vi "Create UNSUBSCRIBE Packet.vi"(5 "UNSUBSCRIBE in":refnum<class "UNSUBSCRIBE.lvclass">, 8 "error in (no error)":errorcluster, 9 "Packet ID (0: generate new)":u16 format="%04x", 11 "Topic Subscriptions":string[](array[string])) -> (0 "error out":errorcluster, 2 "Bytes Stream":u8[](array[numeric]) format="%08b", 3 "UNSUBSCRIBE out":refnum<class "UNSUBSCRIBE.lvclass">)   [LabVIEW 2013, in "MQTT_Control_Packets.lvlib" / "UNSUBSCRIBE.lvclass"]
uses:
  UNSUBSCRIBE.lvclass
  ControlPacket/ControlPacket.lvclass/ControlPacket.ctl
  ControlPacket/ControlPacket.lvclass
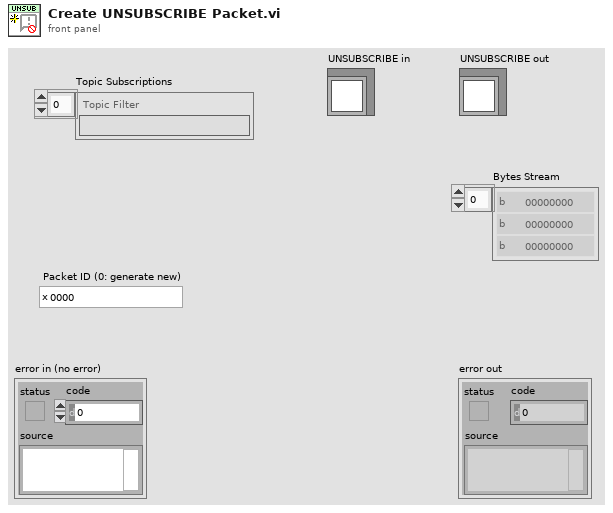
[diagram p1: front panel]
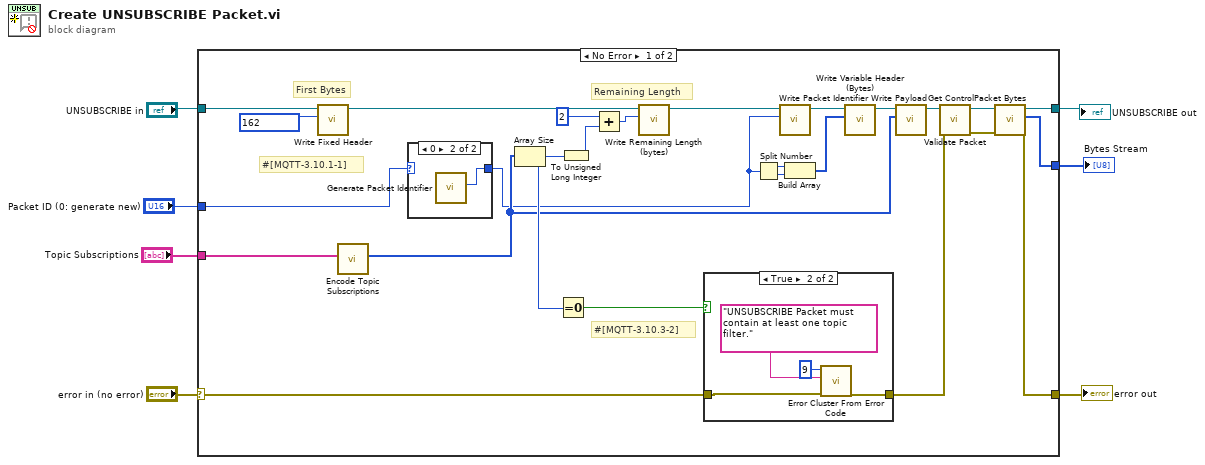
[diagram p0: block diagram]
diagram:
  n1 = case shown="No Error" "error in (no error)" {
    selector: "error in (no error)" -> [w20 w42]
    tunnel: [w9 w42] -> w3
    tunnel: [w11 w41] -> w2
    tunnel: "UNSUBSCRIBE in" -> [w33 w41]
    tunnel: "Packet ID (0: generate new)" -> [w14 _]
    tunnel: "Topic Subscriptions" -> [w16 _]
    tunnel: [w8 _] -> w1
    frame No Error {
      # "#[MQTT-3.10.3-2]"
      # "#[MQTT-3.10.1-1]"
      # "Remaining Length"
      # "First Bytes"
      n2 = call "Write Fixed Header.vi"("Fixed Header"=u8 162, "ControlPacket in"=w33) -> ("ControlPacket out"=w32:refnum<class "UNSUBSCRIBE.lvclass">)  [unwired: 9 in]
      n3 = call "Encode Topic Subscriptions.vi"("Topic Subscriptions"=w16) -> ("Length-Prefixed Field"=w15:u8[])  [unwired: 10 in]
      n4 = case shown="0" w14 {
        selector: w14 -> [w34 _]
        tunnel: [w34 w35] -> w13
        frame Default {
        }
        frame 0 {
          n5 = call "Generate Packet Identifier.vi"() -> ("Packet Identifier"=w35:u16)  [unwired: 11 in]
        }
      }
      n6 = Array Size(array=w15) -> (size(s)=w21:i32)
      n7 = Equal To 0?(x=w21) -> (x = 0?=w19:bool)
      n8 = To Unsigned Long Integer(number=w21) -> (unsigned 32bit integer=w22:u32)
      n9 = Add(x=u32 2 ("Remaining Length (bytes)"), y=w22) -> (x+y=w24:u32)
      n10 = call "Write Remaining Length (bytes).vi"("Remaining Length (bytes)"=w24, "ControlPacket in"=w32) -> ("ControlPacket out"=w28:refnum<class "UNSUBSCRIBE.lvclass">)  [unwired: 9 in]
      n11 = case shown="True" w19 {
        tunnel: w20 -> [w36 w39]
        tunnel: [w36 w40] -> w17
        frame False {
        }
        frame True {
          n12 = call <vilib>:"Error Cluster From Error Code.vi"("error in (no error)"=w39, "error message (\"\")"="UNSUBSCRIBE Packet must contain at least one topic filter.", "error code (0)"=9) -> ("error out"=w40:errorcluster)  [unwired: 6 in]
        }
      }
      n13 = Split Number(x=w13) -> (hi(x)=w31:u8, lo(x)=w30:u8)
      n14 = call "Write Packet Identifier.vi"("Packet Identifier"=w13, "ControlPacket in"=w28) -> ("ControlPacket out"=w27:refnum<class "UNSUBSCRIBE.lvclass">)  [unwired: 9 in]
      n15 = Build Array(w31, w30) -> (w29:u8[])
      n16 = call "Write Variable Header (Bytes).vi"("Variable Header (Bytes)"=w29, "ControlPacket in"=w27) -> ("ControlPacket out"=w23:refnum<class "UNSUBSCRIBE.lvclass">)  [unwired: 9 in]
      n17 = call "Write Payload.vi"("Payload"=w15, "ControlPacket in"=w23) -> ("ControlPacket out"=w18:refnum<class "UNSUBSCRIBE.lvclass">)  [unwired: 9 in]
      n18 = call "Validate Packet.vi"("error in (no error)"=w17, "ControlPacket in"=w18) -> ("error out"=w10:errorcluster, "ControlPacket out"=w12:refnum<class "UNSUBSCRIBE.lvclass">)  [unwired: 8 in]
      n19 = call "Get ControlPacket Bytes.vi"("error in (no error)"=w10, "ControlPacket"=w12) -> ("error out"=w9:errorcluster, "Bytes Stream"=w8:u8[], "ControlPacket dup"=w11:refnum<class "UNSUBSCRIBE.lvclass">)  [unwired: 6 in, 1 out]
    }
    frame Error {
    }
  }
  "error out" <- w3
  "UNSUBSCRIBE out" <- w2
  "Bytes Stream" <- w1
